vi "[ex ce] CSE - Solve system of 2 ODE (R-K method).vi"() -> ()   [LabVIEW 2021]
doc: "This is example of using CalcExpress Script Engine (CSE).\n\nThe example executes a CSE script to solve system of two differential equations using Runge-Kutta method.\n\n::: CalcExpress Toolkit :::\nCopyright (c) 2000-2026 Konstantin Shifershteyn. All rights reserved."
panel:
  out "Solution":cluster{"value out":dbl[], "value out":dbl[]}[](graph)
  in  "y0":dbl=2.0 format="%.2f"
  in  "x0":dbl format="%.2f"
  in  "h":dbl=0.005 format="%#.6f"
  in  "timeEnd":dbl=10.0 format="%.2f"
  in  "timeStart":dbl format="%.2f"
  out "parse time, ms":u32
  in  "stop":bool=TRUE
  in  "abort":bool
  out "exec time, ms":u32
  in  "Script":string="t = timeStart; x = x0; y = y0;     //initial values\nta = nvecifs(timeStart, timeEnd, h);   //time array\nN  = size(ta);                     //number of points\nxa = vectorn(x, N);                //output x values\nya = vectorn(y, N);                //output y values\nxk = yk = vectorn(0,4);            //x and y temporaries\nhk = vector(h/2, h/2, h);          //time coefficients\n\nfor (i=1; i<N; i++ ) {\n  t0=t; x0=x; y0=y;\n  for (j=0; ; j++) {\n    xk[j] = sin(t*x)+y;       // formula 1\n    yk[j] = -t*x-y;           // formula 2\n    if (j >= 3)\n      break;\n    t = t0 + hk[j];\n    x = x0 + xk[j] * hk[j];\n    y = y0 + yk[j] * hk[j];\n  }\n  t = ta[i];\n  xa[i] = x = x0 + h * (xk[0]+2*(xk[1]+xk[2])+xk[3])/6;\n  ya[i] = y = y0 + h * (yk[0]+2*(yk[1]+yk[2])+yk[3])/6;\n}\n"
  # "The script solves a system of two ordinary differential equations using the Runge Kutta method"
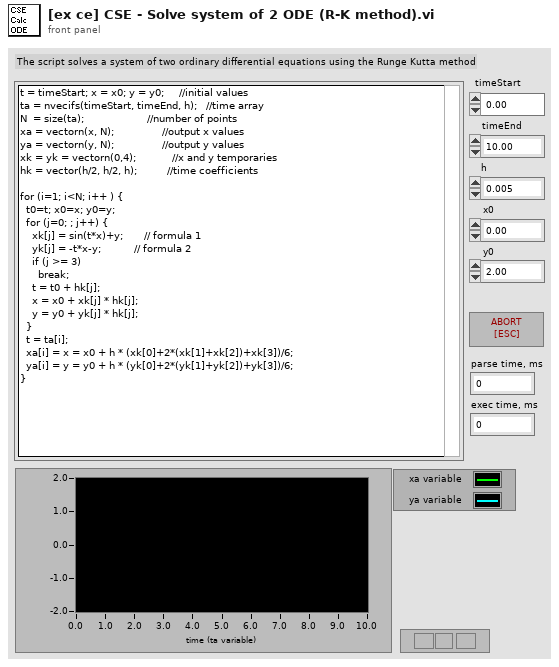
[diagram p1: front panel]
types:
  T1 = typedef "VarMan Variable Context Handle.ctl" = i32
  T2 = enum16{"create", "destroy", "set value", "get value"}
  T3 = typedef "CSE Instance RefNum.ctl" = refnum<k1>
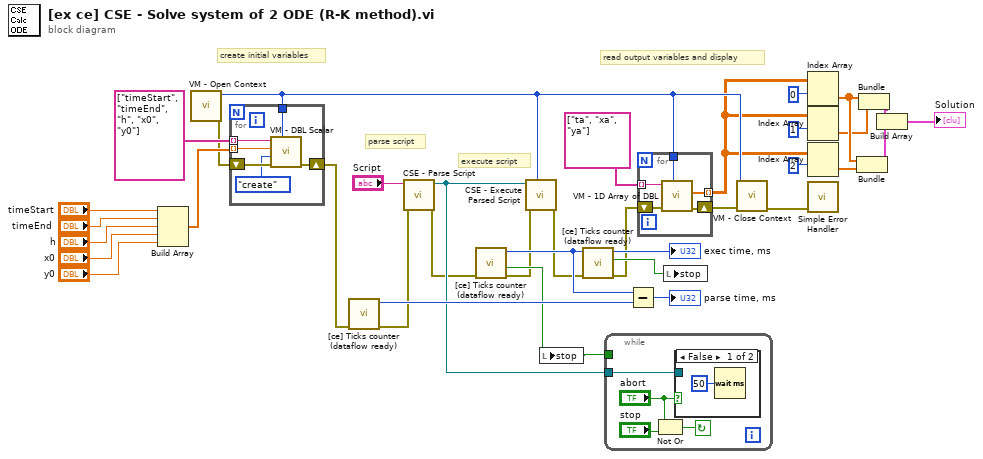
[diagram p0: block diagram]
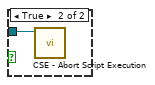
[diagram p2: hidden frame]
diagram:
  # "parse script"
  # "read output variables and display"
  # "execute script"
  # "create initial variables"
  n1 = Build Array("timeStart", "timeEnd", "h", "x0", "y0") -> (w21:dbl[])
  n2 = call "VM - Open Context.vi"() -> ("error out"=w1:errorcluster, "VC Handle out"=w20:T1)  [unwired: 9 in, 1 out]
  n3 = for {
    shift-right: [w42] -> w8
    shift-left: w1 -> [w41]
    tunnel: string[] ["timeStart", "timeEnd", "h", "x0", "y0"] -> [w40] mode=indexing
    tunnel: w20 -> [w39]
    tunnel: w21 -> [w38] mode=indexing
    n4 = call "VM - DBL Scalar.vi"("VC Handle"=w39, "error in"=w41, "cmd"=T2."create", "value in"=w38, "name_spec"=w40) -> ("error out"=w42:errorcluster)  [unwired: 1 in, 5 out]
  }
  n5 = call "[ce] Ticks counter (dataflow ready).vi"("error in"=w8) -> ("error out"=w7:errorcluster, "ticks (current-input)"=w27:u32)  [unwired: 4 in, 3 out]
  n6 = call "CSE - Parse Script.vi"("error in"=w7, "Script"="Script") -> ("error out"=w6:errorcluster, "CSE RefNum"=w23:T3)  [unwired: 5 in, 3 out]
  n7 = call "[ce] Ticks counter (dataflow ready).vi"("error in"=w6) -> ("error out"=w5:errorcluster, "false"=w24:bool, "ticks (current-input)"=w25:u32)  [unwired: 4 in, 2 out]
  n8 = call "CSE - Execute Parsed Script.vi"("VC Handle"=w20, "error in"=w5, "CSE RefNum"=w23) -> ("error out"=w15:errorcluster)  [unwired: 4 in, 4 out]
  n9 = local write "stop"(w24) -> ()
  n10 = call "[ce] Ticks counter (dataflow ready).vi"("error in"=w15, "ticks in"=w25) -> ("error out"=w4:errorcluster, "true"=w30:bool, "ticks (current-input)"=→"exec time, ms":u32)  [unwired: 3 in, 2 out]
  n11 = while {
    tunnel: w24 -> [_]
    tunnel: w23 -> [w46]
    stop <- w44 continue-if-true
    n12 = Not Or(1:"stop", 2:"abort") -> (0:w44:bool)
    n13 = case shown="False" "abort" {
      tunnel: w46 -> [_ w48]
      frame False {
        n14 = Wait (ms)(milliseconds to wait=u32 50) -> ()  [unwired: 1 out]
      }
      frame True {
        n15 = call "CSE - Abort Script Execution.vi"("CSE RefNum"=w48) -> ()  [unwired: 6 in, 3 out]
      }
    }
  }
  n16 = Subtract(x=w25, y=w27) -> (x-y=→"parse time, ms":u32)
  n17 = for {
    tunnel: w20 -> [w53]
    shift-right: [w51] -> w19
    shift-left: w4 -> [w52]
    tunnel: string[] ["ta", "xa", "ya"] -> [w50] mode=indexing
    tunnel: [w49] -> w17 mode=indexing
    n18 = call "VM - 1D Array of DBL.vi"("VC Handle"=w53, "error in"=w52, "name_spec"=w50) -> ("error out"=w51:errorcluster, "value out"=w49:dbl[])  [unwired: 3 in, 4 out]
  }
  n19 = local write "stop"(w30) -> ()
  n20 = call "VM - Close Context.vi"("error in"=w19, "VC Handle"=w20) -> ("error out"=w16:errorcluster)  [unwired: 8 in, 1 out]
  n21 = Index Array(array=w17, index (row)=0) -> (element=w13:dbl[])  [unwired: 1 in]
  n22 = Index Array(array=w17, index (row)=1) -> (element=w3:dbl[])  [unwired: 1 in]
  n23 = Index Array(array=w17, index (row)=2) -> (element=w2:dbl[])  [unwired: 1 in]
  n24 = call <vilib>:"Simple Error Handler.vi"("error in (no error)"=w16) -> ()  [unwired: 4 in, 5 out]
  n25 = Bundle("value out"=w13, "value out"=w2) -> (w12:cluster{"value out":dbl[], "value out":dbl[]})  [unwired: 1 in]
  n26 = Bundle("value out"=w13, "value out"=w3) -> (w14:cluster{"value out":dbl[], "value out":dbl[]})  [unwired: 1 in]
  n27 = Build Array(w14, w12) -> (→"Solution":cluster{"value out":dbl[], "value out":dbl[]}[])
